vi "SLSC Error Suppression.vi"(3 "error in (no error)":errorcluster, 4 "Popup Error?":bool, 5 "Clear All Error?":bool) -> (6 "error?":bool, 10 "error out":errorcluster)   [LabVIEW 2020, in "SLSC CD Shared.lvlib"]
uses:
  SLSC CD Shared.lvlib
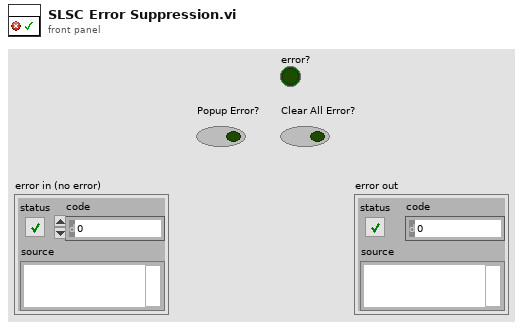
[diagram p1: front panel]
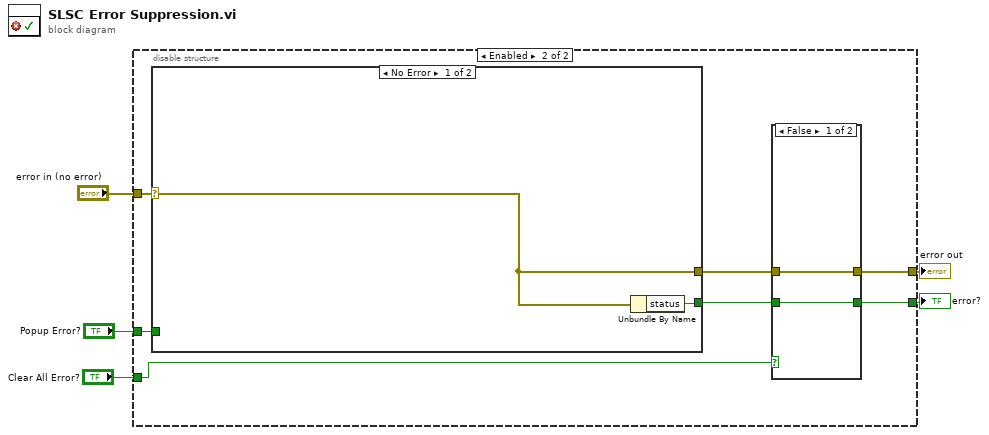
[diagram p0: block diagram]
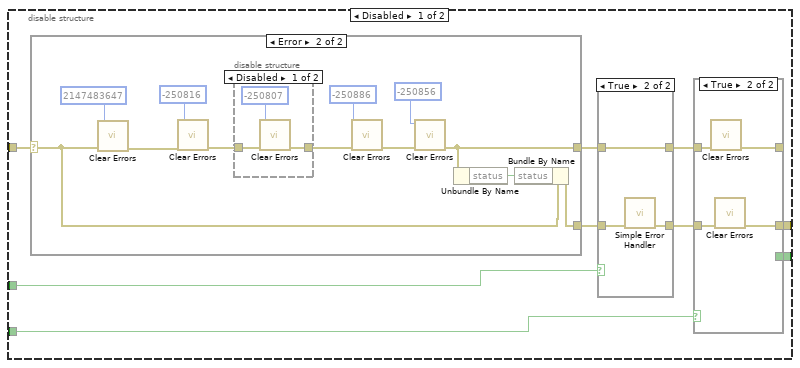
[diagram p2: hidden frame]
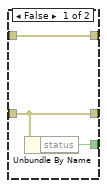
[diagram p3: hidden frame]
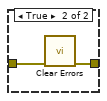
[diagram p7: hidden frame]
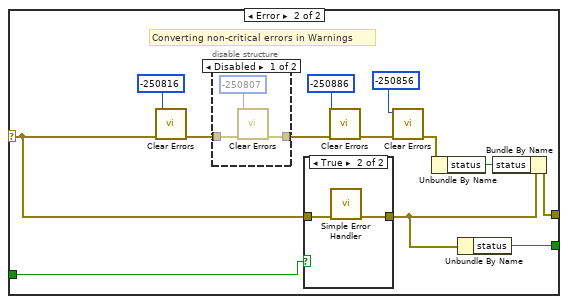
[diagram p8: hidden frame]
diagram:
  n1 = disable-structure shown="Enabled" {
    disable-tunnel: "error in (no error)" -> [w14 w50]
    disable-tunnel: "Popup Error?" -> [w13 w45]
    disable-tunnel: [w11 w48] -> w3
    disable-tunnel: "Clear All Error?" -> [w8 w46]
    disable-tunnel: [w6 w47] -> w1
    frame Disabled {
      n2 = case shown="Error" w14 {
        selector: w14 -> [w27 w28]
        tunnel: [w27 w31] -> w10
        tunnel: [w27 w29] -> w7
        frame No Error {
        }
        frame Error {
          n3 = call <vilib>:"Clear Errors.vi"("error in (no error)"=w28, "specific error code to clear (0: all)"=2147483647) -> ("error out"=w32:errorcluster)  [unwired: 4 in, 1 out]
          n4 = call <vilib>:"Clear Errors.vi"("error in (no error)"=w32, "specific error code to clear (0: all)"=-250816) -> ("error out"=w38:errorcluster)  [unwired: 4 in, 1 out]
          n5 = disable-structure shown="Disabled" {
            disable-tunnel: w38 -> [w41 w43]
            disable-tunnel: [w40 w43] -> w39
            frame Disabled {
              n6 = call <vilib>:"Clear Errors.vi"("error in (no error)"=w41, "specific error code to clear (0: all)"=-250807) -> ("error out"=w40:errorcluster)  [unwired: 4 in, 1 out]
            }
            frame Enabled {
            }
          }
          n7 = call <vilib>:"Clear Errors.vi"("error in (no error)"=w39, "specific error code to clear (0: all)"=-250886) -> ("error out"=w35:errorcluster)  [unwired: 4 in, 1 out]
          n8 = call <vilib>:"Clear Errors.vi"("error in (no error)"=w35, "specific error code to clear (0: all)"=-250856) -> ("error out"=w31:errorcluster)  [unwired: 4 in, 1 out]
          n9 = Unbundle By Name(w31) -> ("status"=w30:bool)
          n10 = Bundle By Name(cluster=w28, "status"=w30) -> (w29:errorcluster)
        }
      }
      n11 = case shown="True" w13 {
        tunnel: w7 -> [w23 w26]
        tunnel: [w23 w25] -> w12
        tunnel: [w22 w24] -> w9
        tunnel: w10 -> [w22 w24]
        frame False {
        }
        frame True {
          n12 = call <vilib>:"Simple Error Handler.vi"("error in (no error)"=w26) -> ("error out"=w25:errorcluster)  [unwired: 4 in, 4 out]
        }
      }
      n13 = case shown="True" w8 {
        tunnel: w12 -> [w16 w21]
        tunnel: [w16 w20] -> w11
        tunnel: w9 -> [w17 w19]
        tunnel: [w17 w18] -> _
        tunnel: [w15 _] -> w6
        frame False {
          n14 = Unbundle By Name(w16) -> ("status"=w15:bool)
        }
        frame True {
          n15 = call <vilib>:"Clear Errors.vi"("error in (no error)"=w19) -> ("error out"=w18:errorcluster)  [unwired: 5 in, 1 out]
          n16 = call <vilib>:"Clear Errors.vi"("error in (no error)"=w21) -> ("error out"=w20:errorcluster)  [unwired: 5 in, 1 out]
        }
      }
    }
    frame Enabled {
      n17 = case shown="No Error" w50 {
        selector: w50 -> [w55 w60]
        tunnel: [w55 w61] -> w49
        tunnel: w45 -> [_ w59]
        tunnel: [w56 w57] -> w44
        frame No Error {
          n18 = Unbundle By Name(w55) -> ("status"=w56:bool)
        }
        frame Error {
          # "Converting non-critical errors in Warnings"
          n19 = call <vilib>:"Clear Errors.vi"("error in (no error)"=w60, "specific error code to clear (0: all)"=-250816) -> ("error out"=w68:errorcluster)  [unwired: 4 in, 1 out]
          n20 = disable-structure shown="Disabled" {
            disable-tunnel: w68 -> [w74 w76]
            disable-tunnel: [w73 w76] -> w69
            frame Disabled {
              n21 = call <vilib>:"Clear Errors.vi"("error in (no error)"=w74, "specific error code to clear (0: all)"=-250807) -> ("error out"=w73:errorcluster)  [unwired: 4 in, 1 out]
            }
            frame Enabled {
            }
          }
          n22 = case shown="True" w59 {
            tunnel: w60 -> [w70 w72]
            tunnel: [w70 w71] -> w58
            frame False {
            }
            frame True {
              n23 = call <vilib>:"Simple Error Handler.vi"("error in (no error)"=w72) -> ("error out"=w71:errorcluster)  [unwired: 4 in, 4 out]
            }
          }
          n24 = call <vilib>:"Clear Errors.vi"("error in (no error)"=w69, "specific error code to clear (0: all)"=-250886) -> ("error out"=w65:errorcluster)  [unwired: 4 in, 1 out]
          n25 = call <vilib>:"Clear Errors.vi"("error in (no error)"=w65, "specific error code to clear (0: all)"=-250856) -> ("error out"=w63:errorcluster)  [unwired: 4 in, 1 out]
          n26 = Unbundle By Name(w63) -> ("status"=w62:bool)
          n27 = Unbundle By Name(w58) -> ("status"=w57:bool)
          n28 = Bundle By Name(cluster=w58, "status"=w62) -> (w61:errorcluster)
        }
      }
      n29 = case shown="False" w46 {
        tunnel: w49 -> [w52 w54]
        tunnel: [w52 w53] -> w48
        tunnel: [w51 _] -> w47
        tunnel: w44 -> [w51 _]
        frame False {
        }
        frame True {
          n30 = call <vilib>:"Clear Errors.vi"("error in (no error)"=w54) -> ("error out"=w53:errorcluster)  [unwired: 5 in, 1 out]
        }
      }
    }
  }
  "error out" <- w3
  "error?" <- w1
